vi "Sequence.BuildPreviewiStep.vi"(8 "Step":T1, 9 "Step IO":cluster{"Ramp Pattern":dbl[]}, 10 "iStep Iterations":i32, 11 "Step Duration":u64) -> (3 "Ramp Pattern":dbl[](array[numeric]))   [LabVIEW 2015, in "Simple Sequence Tools - Shared.lvlib"]
uses:
  Simple Sequence Tools - Shared.lvlib
  Types/Step.Types.ctl
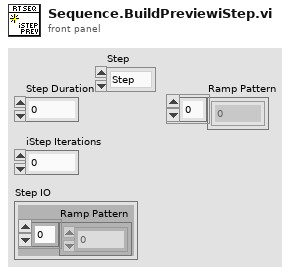
[diagram p1: front panel]
types:
  T1 = typedef "Simple Sequence Tools - Shared.lvlib/Step.Types.ctl" = enum8{"Step", "iStep", "Ramp", "Unchanged", "Unknown", "Sine", "LogSine", "LinearSine", "ForcedRamp", "SquareWave"}
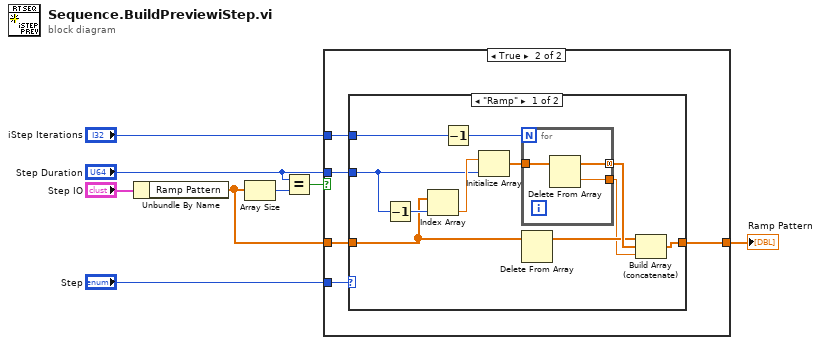
[diagram p0: block diagram]
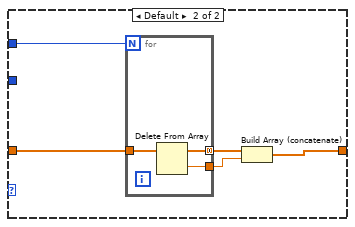
[diagram p3: hidden frame]
diagram:
  n1 = Unbundle By Name("Step IO") -> ("Ramp Pattern"=w6:dbl[])
  n2 = Array Size(array=w6) -> (size(s)=w2:i32)
  n3 = Equal?(x="Step Duration", y=w2) -> (x = y?=w7:bool)
  n4 = case shown="True" w7 {
    tunnel: "iStep Iterations" -> [_ w14]
    tunnel: w6 -> [w9 w13]
    tunnel: [w9 w12] -> w8
    tunnel: "Step" -> [_ w11]
    tunnel: "Step Duration" -> [_ w10]
    frame False {
    }
    frame True {
      n5 = case shown="\"Ramp\"" w11 {
        tunnel: w14 -> [w25 w33]
        tunnel: w13 -> [w17 w32]
        tunnel: [w19 w30] -> w12
        tunnel: w10 -> [w18 _]
        frame "Ramp" {
          n6 = Decrement(x=w18) -> (x-1=w23:u64)
          n7 = Index Array(array=w17, index=w23) -> (element=w22:dbl)
          n8 = Decrement(x=w25) -> (x-1=w24:i32)
          n9 = Initialize Array(w22, w18) -> (w21:dbl[])
          n10 = for {
            N: w24 -> [_]
            tunnel: w21 -> [w28]
            tunnel: [w27] -> w20 mode=concatenating
            tunnel: [w26] -> w15
            n11 = Delete From Array(array=w28) -> (deleted portion=w26:dbl, array with subset deleted=w27:dbl[])  [unwired: 2 in]
          }
          n12 = Delete From Array(array=w17) -> (array with subset deleted=w16:dbl[])  [unwired: 2 in, 1 out]
          n13 = Build Array (concatenate)(w16, w20, w15) -> (w19:dbl[])
        }
        frame Default {
          n14 = for {
            N: w33 -> [_]
            tunnel: w32 -> [w36]
            tunnel: [w35] -> w31 mode=concatenating
            tunnel: [w34] -> w29
            n15 = Delete From Array(array=w36) -> (deleted portion=w34:dbl, array with subset deleted=w35:dbl[])  [unwired: 2 in]
          }
          n16 = Build Array (concatenate)(w31, w29) -> (w30:dbl[])
        }
      }
    }
  }
  "Ramp Pattern" <- w8
